vi "RDC-water-generate_parameter.vi"() -> (3 "parameter map":map{i32, T1}(c390))   [LabVIEW 2020, in "RDC-Reflection_Data_Computation.lvlib"]
doc: "Builds a map of water model parameters per temperature (eps s, eps infi, tau) by interpolating the table from RDC-water-read_parameter."
uses:
  RDC-Reflection_Data_Computation.lvlib
  RDC-water-param.ctl
  <vilib>/gmath/NI_Gmath.lvlib
panel:
  out "temp":dbl[](array[numeric])
  out "temp used":dbl[][](array[numeric])
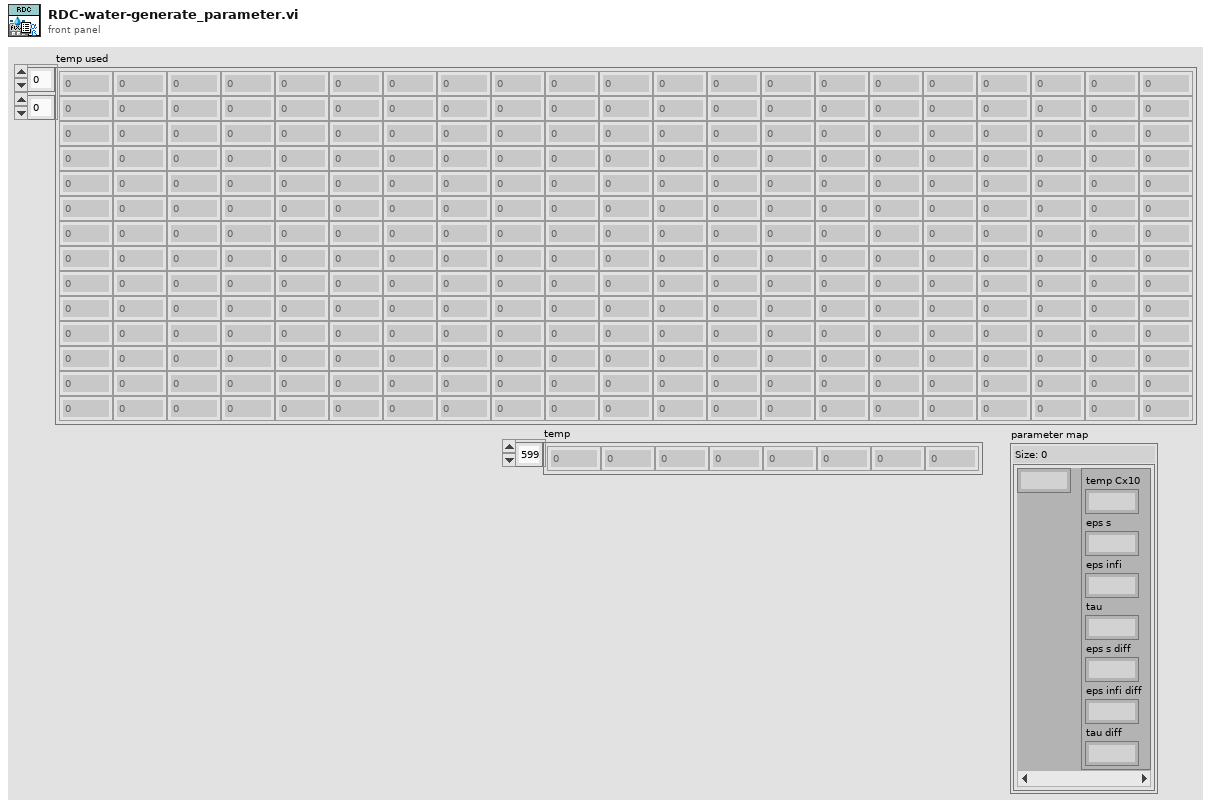
[diagram p1: front panel]
types:
  T1 = typedef "RDC-Reflection_Data_Computation.lvlib/RDC-water-param.ctl" = cluster{"temp Cx10":u16, "eps s":dbl, "eps infi":dbl, "tau":dbl, "eps s diff":dbl, "eps infi diff":dbl, "tau diff":dbl}
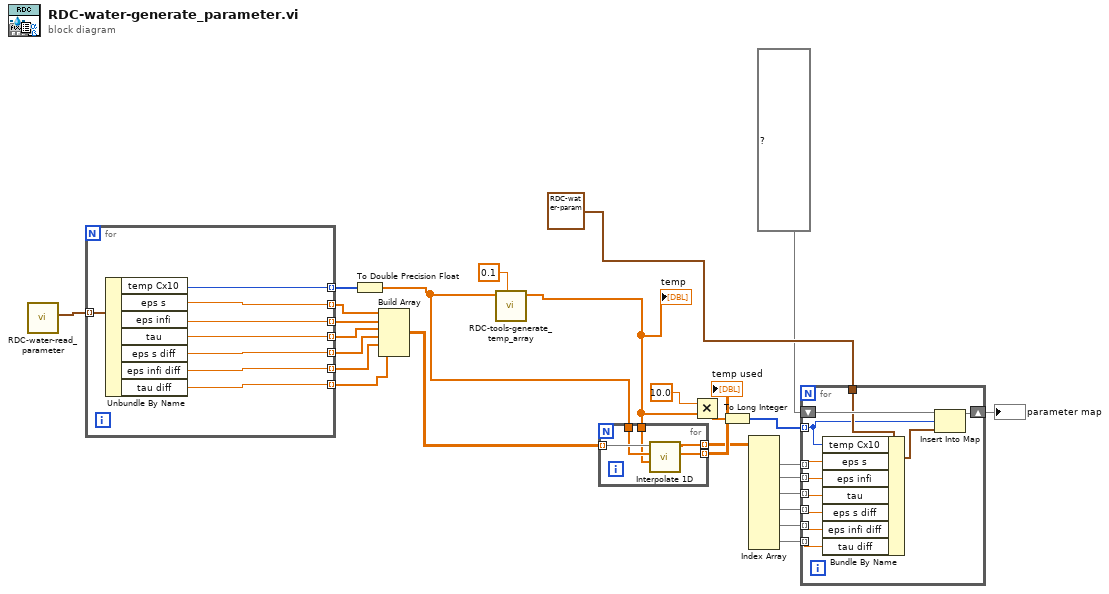
[diagram p0: block diagram]
diagram:
  n1 = call "RDC-water-read_parameter.vi"() -> ("water param Array"=w26:T1[])  [unwired: 10 in, 1 out]
  n2 = for {
    tunnel: w26 -> [w34] mode=indexing
    tunnel: [w33] -> w24 mode=indexing
    tunnel: [w32] -> w23 mode=indexing
    tunnel: [w31] -> w22 mode=indexing
    tunnel: [w30] -> w21 mode=indexing
    tunnel: [w29] -> w19 mode=indexing
    tunnel: [w28] -> w18 mode=indexing
    tunnel: [w27] -> w17 mode=indexing
    n3 = Unbundle By Name(w34) -> ("temp Cx10"=w30:u16, "eps s"=w33:dbl, "eps infi"=w32:dbl, "tau"=w31:dbl, "eps s diff"=w29:dbl, "eps infi diff"=w28:dbl, "tau diff"=w27:dbl)
  }
  n4 = To Double Precision Float(number=w21) -> (double precision float=w3:dbl[])
  n5 = Build Array(w24, w23, w22, w19, w18, w17) -> (w25:dbl[][])
  n6 = call "RDC-tools-generate_temp_array.vi"("Increment"=0.1 ("y"), "temp Cx10"=w3) -> ("temp C"=w2:dbl[])  [unwired: 9 in]
  "temp" <- w2
  n7 = for {
    tunnel: w25 -> [w39] mode=indexing
    tunnel: [w38] -> w16 mode=indexing
    tunnel: w3 -> [w37]
    tunnel: w2 -> [w35]
    tunnel: [w36] -> w20 mode=indexing
    n8 = call <vilib>:"Interpolate 1D.vi"("xi"=w35, "X"=w37, "Y"=w39) -> ("xi used"=w36:dbl[], "yi"=w38:dbl[])  [unwired: 6 in, 1 out]
  }
  "temp used" <- w20
  n9 = Multiply(x=10.0 ("temp C"), y=w2) -> (x*y=w6:dbl[])
  n10 = To Long Integer(number=w6) -> (32bit integer=w15:i32[])
  n11 = Index Array(array=w16) -> (element #1=w14:dbl[], element #2=w13:dbl[], element #3=w12:dbl[], element #4=w11:dbl[], element #5=w10:dbl[], element #6=w9:dbl[])  [unwired: 12 in]
  n12 = for {
    tunnel: w15 -> [w47] mode=indexing
    tunnel: w14 -> [w41] mode=indexing
    tunnel: w13 -> [w42] mode=indexing
    tunnel: w12 -> [w43] mode=indexing
    tunnel: w11 -> [w44] mode=indexing
    tunnel: w10 -> [w45] mode=indexing
    tunnel: w9 -> [w46] mode=indexing
    shift-right: [w40] -> w7
    shift-left: map{i32, T1} {} ("map") -> [w50]
    tunnel: T1 {"temp Cx10"=250, "eps s"=78.36, "eps infi"=5.2, "tau"=8.27e-12, "eps s diff"=78.36, "eps infi diff"=5.2, "tau diff"=8.27e-12} ("water values") -> [w49]
    n13 = Bundle By Name(cluster=w49, "temp Cx10"=w47, "eps s"=w41, "eps infi"=w42, "tau"=w43, "eps s diff"=w44, "eps infi diff"=w45, "tau diff"=w46) -> (w48:T1)
    n14 = Insert Into Map(map in=w50, key=w47, value=w48) -> (map out=w40:map{i32, T1})  [unwired: 2 out]
  }
  "parameter map" <- w7
